vi "Function VI Template.vi"(8 "error in":errorcluster, 11 "Input Parameters":cluster{}) -> (0 "error out":errorcluster, 3 "Output Parameters":cluster{})   [LabVIEW 2026]
uses:
  Type Definitions/Type Definition Template--cluster.ctl
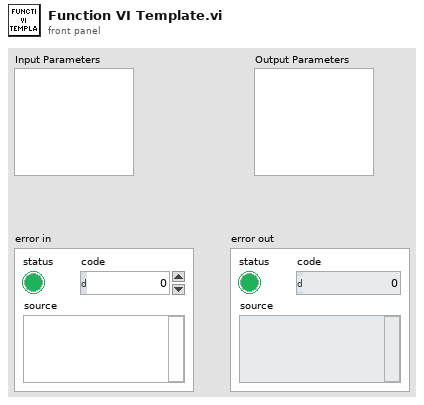
[diagram p1: front panel]
types:
  T1 = typedef "Type Definition Template--cluster.ctl" = cluster{}
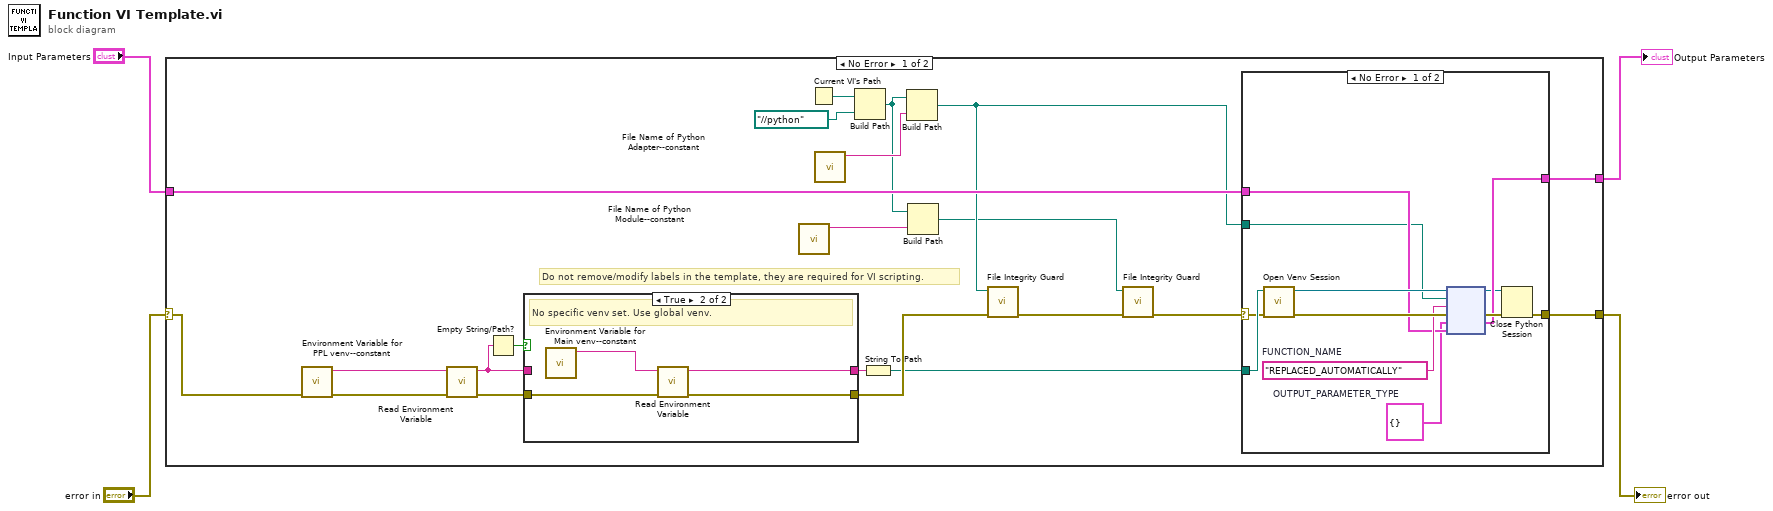
[diagram p0: block diagram]
diagram:
  n1 = case shown="No Error" "error in" {
    selector: "error in" -> [w22 w45]
    tunnel: "Input Parameters" -> [w17 _]
    tunnel: [w16 _] -> w1
    tunnel: [w23 w45] -> w4
    frame No Error {
      # "Do not remove/modify labels in the template, they are required for VI scripting."
      n2 = call "Environment Variable for PPL venv--constant.vi"("error in"=w22) -> ("error out"=w25:errorcluster, "Environment Variable for Main venv"=w21:string)  [unwired: 9 in]
      n3 = call "Read Environment Variable.vi"("error in"=w25, "Variable"=w21) -> ("error out"=w24:errorcluster, "Value"=w18:string)  [unwired: 8 in]
      n4 = Empty String/Path?(string/path=w18) -> (empty?=w20:bool)
      n5 = case shown="True" w20 {
        tunnel: w24 -> [w40 w44]
        tunnel: [w39 w41] -> w19
        tunnel: [w40 w43] -> w13
        tunnel: w18 -> [w39 _]
        frame False {
          # "Specific venv found."
        }
        frame True {
          # "No specific venv set. Use global venv."
          n6 = call "Environment Variable for Main venv--constant.vi"() -> ("Environment Variable for Main venv"=w42:string)  [unwired: 11 in]
          n7 = call "Read Environment Variable.vi"("error in"=w44, "Variable"=w42) -> ("error out"=w43:errorcluster, "Value"=w41:string)  [unwired: 8 in]
        }
      }
      n8 = call "File Name of Python Module--constant.vi"() -> ("File Name of Python Module"=w6:string)  [unwired: 11 in]
      n9 = Current VI's Path() -> (path=w11:path)
      n10 = call "File Name of Python Adapter--constant.vi"() -> ("File Name of Python Adapter"=w15:string)  [unwired: 11 in]
      n11 = Build Path(base path=w11, name or relative path=path "../../python") -> (appended path=w7:path)
      n12 = String To Path(string=w19) -> (path=w12:path)
      n13 = Build Path(base path=w7, name or relative path=w15) -> (appended path=w14:path)
      n14 = Build Path(base path=w7, name or relative path=w6) -> (appended path=w5:path)
      n15 = call "File Integrity Guard.vi"("error in"=w13, "File Path"=w14) -> ("error out"=w9:errorcluster)  [unwired: 9 in]
      n16 = call "File Integrity Guard.vi"("error in"=w9, "File Path"=w5) -> ("error out"=w8:errorcluster)  [unwired: 9 in]
      n17 = case shown="No Error" w8 {
        selector: w8 -> [w26 w38]
        tunnel: [w35 w38] -> w23
        tunnel: w17 -> [w32 _]
        tunnel: [w31 _] -> w16
        tunnel: w14 -> [w28 _]
        tunnel: w12 -> [w27 _]
        frame No Error {
          w29 = T1 {}  # OUTPUT_PARAMETER_TYPE
          w33 = "REPLACED_AUTOMATICALLY"  # FUNCTION_NAME
          n18 = call "Open Venv Session.vi"("error in"=w26, "Venv"=w27) -> ("error out"=w37:errorcluster, "session out"=w34:refnum<k35>)  [unwired: 8 in]
          n19 = node(w34, w28, w33, w37, w29, w32) -> (w30:refnum<k35>, w36:errorcluster, w31:T1)  [unwired: 1 in, 2 out]
          n20 = Close Python Session(session in=w30, error in=w36) -> (11:w35:errorcluster)
        }
        frame Error {
          # "Suppres running code if integrity check fails."
        }
      }
    }
    frame Error {
      # "Pass error without any actions."
    }
  }
  "error out" <- w4
  "Output Parameters" <- w1
